vi "Cache Hints.vi"(11 "method":string) -> (1 "cacheable?":bool, 2 "cacheScope":string, 3 "ttlMs":i32)   [LabVIEW 2020, in "MCP Server.lvlib"]
doc: "The caching hints (ttlMs and cacheScope) that modern (MCP 2026-07-28) results carry, kept in one place.\n\n- server/discover, tools/list, prompts/list, resources/list and resources/templates/list: ttlMs 60000, cacheScope \"public\". What these answer only changes when the application adds tools, prompts or resources, which a toolkit server normally does once at start, so a client may reuse the answer for a minute. It is \"public\" because the answer is the same for every client: the server has no users or sessions.\n- resources/read: ttlMs 0, cacheScope \"public\". A file resource is read from disk on every request and the file can change at any time, so it must not be reused; it is still the same for every client.\n- Every other method: cacheable? is FALSE and the result gets neither field (the spec requires them only on the methods above, and never on input_required results)."
uses:
  MCP Server.lvlib
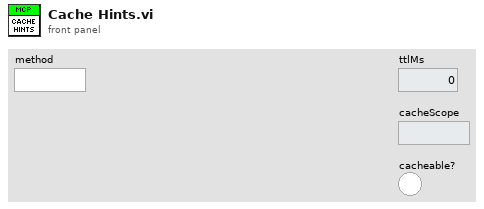
[diagram p1: front panel]
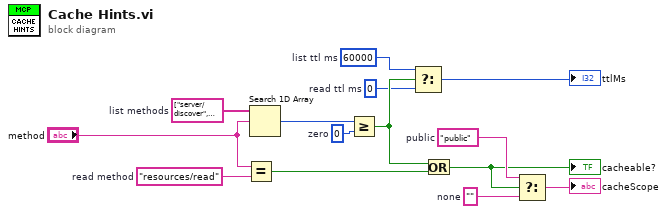
[diagram p0: block diagram]
diagram:
  w12 = 0  # zero
  w4 = ""  # none
  w5 = "public"  # public
  w6 = 0  # read ttl ms
  w8 = 60000  # list ttl ms
  w10 = "resources/read"  # read method
  w14 = string[] ["server/discover", "tools/list", "prompts/list", "resources/list", "resources/templates/list"]  # list methods
  n1 = Equal?(x="method", y=w10) -> (x = y?=w9:bool)
  n2 = Search 1D Array(1D array=w14, element="method") -> (index of element=w13:i32)  [unwired: 1 in]
  n3 = Greater Or Equal?(x=w13, y=w12) -> (x >= y?=w7:bool)
  n4 = Select(t=w8, s=w7, f=w6) -> (s? t:f=→"ttlMs":i32)
  n5 = Or(x=w7, y=w9) -> (x .or. y?=w1:bool)
  "cacheable?" <- w1
  n6 = Select(t=w5, s=w1, f=w4) -> (s? t:f=→"cacheScope":string)
